vi "get TurnTable Parameter.vi"(8 "error in (no error)":errorcluster caption="에러 입력(에러 없음)", 11 "AUDIX EM1000 입력":refnum<class "AUDIX EM1000.lvclass">) -> (0 "error out":errorcluster caption="에러 출력", 2 "Turn Table Info":T1 {"Target Angle" min=0.0 max=360.0}, 3 "AUDIX EM1000 출력":refnum<class "AUDIX EM1000.lvclass">)   [LabVIEW 2023, in "Turn Table and Mast.lvlib" / "AUDIX EM1000.lvclass"]
uses:
  AUDIX EM1000.lvclass
  AUDIX EM1000.lvclass/AUDIX EM1000.ctl
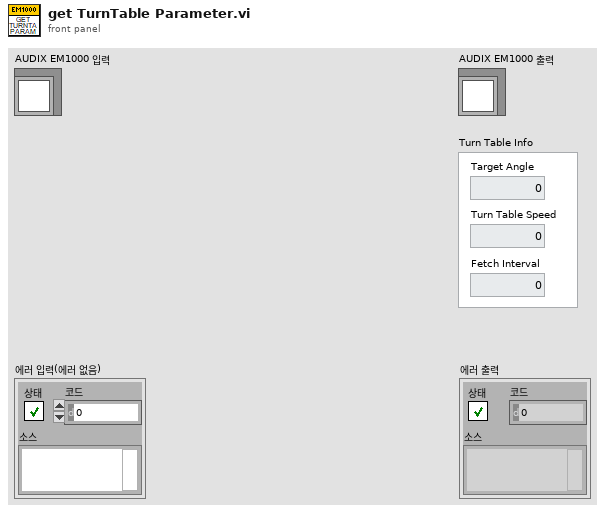
[diagram p1: front panel]
types:
  T1 = cluster{"Target Angle":dbl, "Turn Table Speed":i32, "Fetch Interval":i32}
  T2 = cluster{"Target Angle":dbl, "Speed":i32, "Fetch Interval":i32}
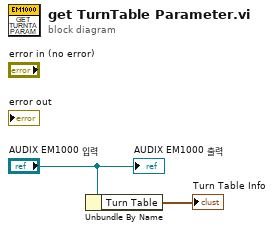
[diagram p0: block diagram]
diagram:
  n1 = Unbundle By Name("AUDIX EM1000 입력") -> ("Turn Table"=→"Turn Table Info":T2)
  "AUDIX EM1000 출력" <- "AUDIX EM1000 입력"
